vi "Filter.vi"(8 "error in (no error)":errorcluster, 10 "Selected Runnables":string[](array[string]), 11 "LUnit Test Suite In":refnum<class "LUnit Test Suite.lvclass">) -> (0 "error out":errorcluster, 3 "LUnit Test Suite Out":refnum<class "LUnit Test Suite.lvclass">)   [LabVIEW 2020, in "LUnit Test Suite.lvclass"]
doc: "Select which tests are active. This applies recursively to nested suites."
uses:
  LUnit Test Suite.lvclass
  C:/git/astemes-lunit/source/Runnable.lvclass
  LUnit Test Suite.lvclass/LUnit Test Suite.ctl
  Runnable.lvclass
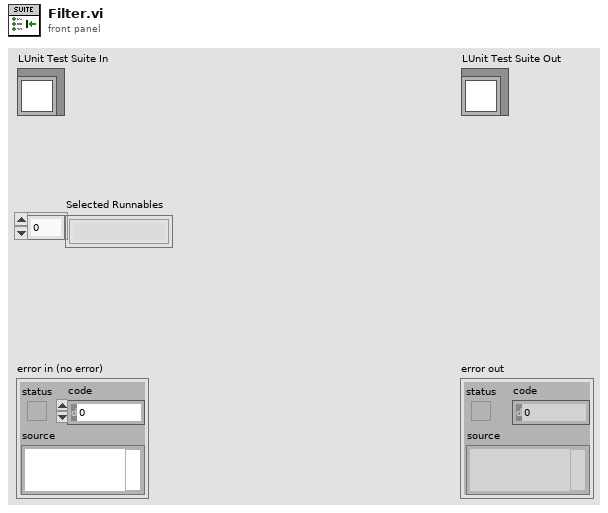
[diagram p1: front panel]
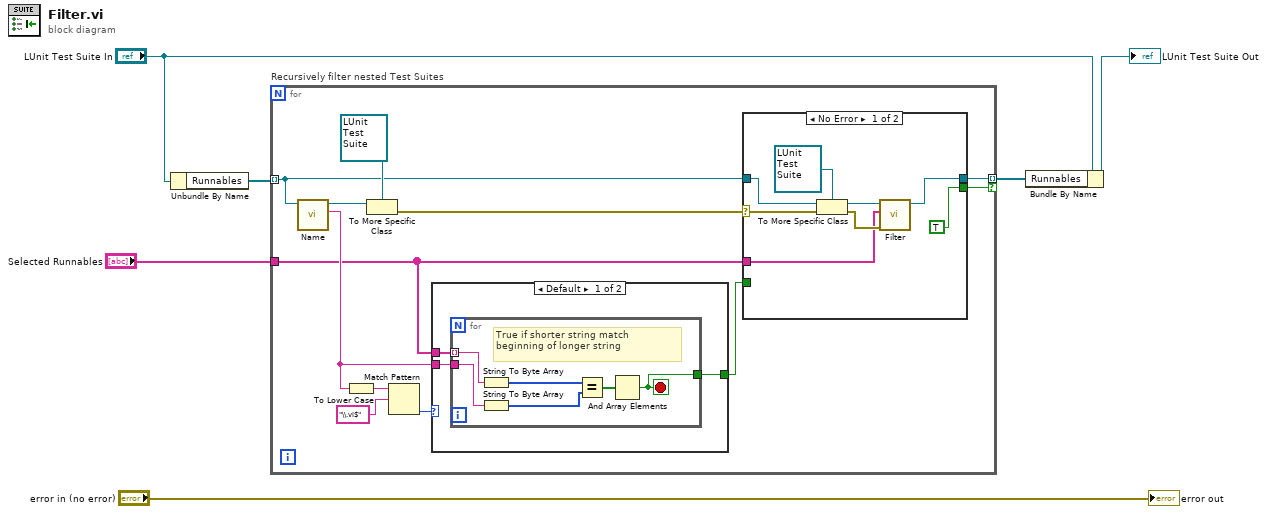
[diagram p0: block diagram]
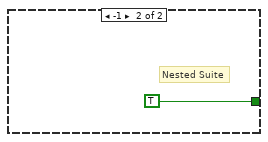
[diagram p2: hidden frame]
diagram:
  n1 = Unbundle By Name("LUnit Test Suite In") -> ("Runnables"=w2:refnum<class "Runnable.lvclass">[])
  n2 = for "Recursively filter nested Test Suites" {
    tunnel: "Selected Runnables" -> [w7]
    tunnel: w2 -> [w10] mode=indexing
    tunnel: [w9] -> w1 mode=indexing if=w8
    n3 = call-dynamic "Name.vi"("Runnable in"=w10) -> ("Name"=w11:string, "Runnable out"=w12:refnum<class "Runnable.lvclass">)  [unwired: 8 in, 1 out]
    n4 = To Lower Case(string=w11) -> (all lower case string=w15:string)
    n5 = To More Specific Class(target class=refnum<class "LUnit Test Suite.lvclass"> refnum ("LUnit Test Suite V2.lvclass"), reference=w12) -> (error out=w17:errorcluster)  [unwired: 1 in, 1 out]
    n6 = Match Pattern(string=w15, regular expression="\\.vi$") -> (offset past match=w14:i32)  [unwired: 1 in, 3 out]
    n7 = case shown="Default" w14 {
      tunnel: w7 -> [w21 _]
      tunnel: [w20 TRUE] -> w16
      tunnel: w11 -> [w19 _]
      frame Default {
        n8 = for {
          tunnel: w21 -> [w27] mode=indexing
          tunnel: w19 -> [w26]
          tunnel: [w22] -> w20
          stop <- w22 stop-if-true
          # "True if shorter string match beginning of longer string"
          n9 = String To Byte Array(string=w27) -> (unsigned byte array=w25:u8[])
          n10 = String To Byte Array(string=w26) -> (unsigned byte array=w24:u8[])
          n11 = Equal?(x=w25, y=w24) -> (x = y?=w23:bool[])
          n12 = And Array Elements(Boolean array=w23) -> (logical AND=w22:bool)
        }
      }
      frame -1 {
        # "Nested Suite"
      }
    }
    n13 = case shown="No Error" w17 {
      selector: w17 -> [w34 _]
      tunnel: w10 -> [w35 w38]
      tunnel: [w31 w38] -> w9
      tunnel: w7 -> [w30 _]
      tunnel: w16 -> [_ w37]
      tunnel: [TRUE w37] -> w8
      frame No Error {
        n14 = To More Specific Class(target class=refnum<class "LUnit Test Suite.lvclass"> refnum ("LUnit Test Suite V2.lvclass"), reference=w35, error in=w34) -> (specific class reference=w33:refnum<class "LUnit Test Suite.lvclass">, error out=w32:errorcluster)
        n15 = call "Filter.vi"("error in (no error)"=w32, "Selected Runnables"=w30, "LUnit Test Suite In"=w33) -> ("LUnit Test Suite Out"=w31:refnum<class "LUnit Test Suite.lvclass">)  [unwired: 7 in, 1 out]
      }
      frame Error {
      }
    }
  }
  n16 = Bundle By Name(cluster="LUnit Test Suite In", "Runnables"=w1) -> (→"LUnit Test Suite Out":refnum<class "LUnit Test Suite.lvclass">)
  "error out" <- "error in (no error)"
